vi "Handle Last Ack.vi"(8 "error in (no error)":errorcluster, 10 "Volatus:Module":refnum<class "Module.lvclass">, 11 "Volatus Core in":refnum<class "Volatus Core.lvclass">) -> (0 "error out":errorcluster, 3 "Volatus Core out":refnum<class "Volatus Core.lvclass">)   [LabVIEW 2020, in "Volatus.lvlib" / "Volatus Core.lvclass"]
uses:
  Volatus Core.lvclass
  C:/dev/lv20CE/relink/lv-volatus/Volatus/Module/Module.lvclass
  Module/Module.lvclass
  Reload State.ctl
  Volatus Core.lvclass/Volatus Core.ctl
  Module/Module.lvclass/Module.ctl
  MessageQ/MessageQ.lvclass/MessageQ.ctl
  Module/Self Q.vi
  MessageQ/Send.vi
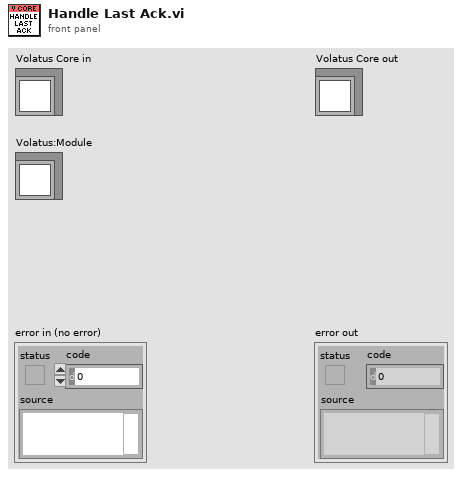
[diagram p1: front panel]
types:
  T1 = typedef "Volatus.lvlib/Volatus Core.lvclass/Reload State.ctl" = enum16{"None", "Stop Modules", "Close Vecto", "Reload", "Restart"}
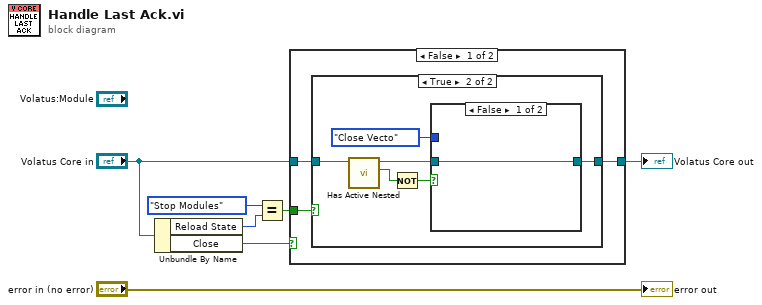
[diagram p0: block diagram]
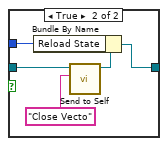
[diagram p3: hidden frame]
diagram:
  n1 = Unbundle By Name("Volatus Core in") -> ("Reload State"=w6:T1, "Close"=w1:bool)
  n2 = Equal?(x=Reload_State."Stop Modules", y=w6) -> (x = y?=w3:bool)
  n3 = case shown="False" w1 {
    tunnel: "Volatus Core in" -> [w8 w24]
    tunnel: w3 -> [w10 _]
    tunnel: [w9 w24] -> w2
    frame False {
      n4 = case shown="True" w10 {
        tunnel: w8 -> [w11 w17]
        tunnel: [w11 w15] -> w9
        frame False {
        }
        frame True {
          n5 = call "Has Active Nested.vi"("Module in"=w17) -> ("Has Active Nested"=w13:bool, "Module out"=w14:refnum<class "Volatus Core.lvclass">)  [unwired: 8 in, 1 out]
          n6 = Not(x=w13) -> (.not. x?=w12:bool)
          n7 = case shown="False" w12 {
            tunnel: w14 -> [w18 w23]
            tunnel: Reload_State."Close Vecto" ("Reload State") -> [_ w21]
            tunnel: [w18 w20] -> w15
            frame False {
            }
            frame True {
              n8 = call "Send to Self.vi"("Message ID"="Close Vecto", "Module in"=w23) -> ("Module out"=w22:refnum<class "Volatus Core.lvclass">)  [unwired: 8 in, 1 out]
              n9 = Bundle By Name(cluster=w22, "Reload State"=w21) -> (w20:refnum<class "Volatus Core.lvclass">)
            }
          }
        }
      }
    }
    frame True {
    }
  }
  "Volatus Core out" <- w2
  "error out" <- "error in (no error)"
